vi "FuncVI_Sub - XYGraph - Master.vi"() -> ()   [LabVIEW 2021]
doc: "::: CalcExpress Toolkit :::\nCopyright (c) 2000-2026 Konstantin Shifershteyn. All rights reserved."
panel:
  in  "data":string
  in  "update":bool
  out "graph":T1(graph)
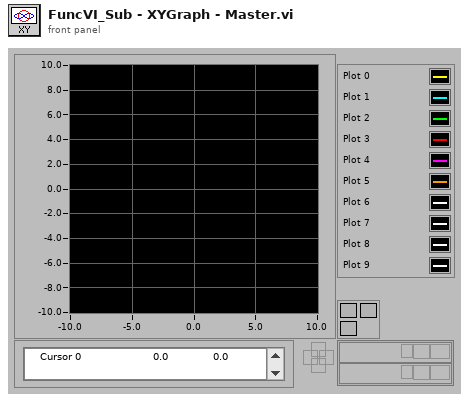
[diagram p1: front panel]
types:
  T1 = cluster{"Sine Wave":dbl[], "Sine Wave copy":dbl[]}[]
  T2 = typedef "LVRectTypeDef.ctl" = cluster{"Left":i16, "Top":i16, "Right":i16, "Bottom":i16}
  T3 = cluster{"plot":i32, "X":dbl[], "Y":dbl[], "plot name":string}
  T4 = cluster{"Sine Wave":dbl[], "Sine Wave copy":dbl[]}
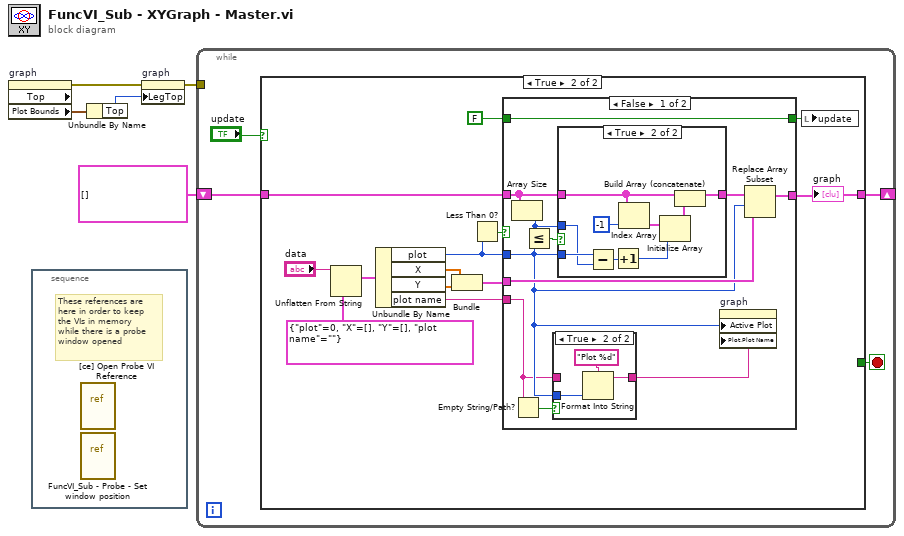
[diagram p0: block diagram]
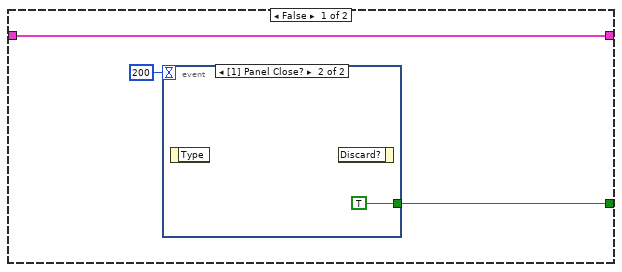
[diagram p2: hidden frame]
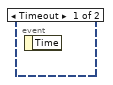
[diagram p3: hidden frame]
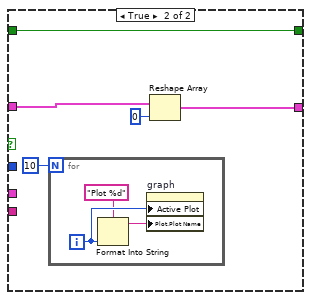
[diagram p6: hidden frame]
diagram:
  n1 = property on="graph" class="XYGraph (strict)" props=["Top", "Plot Bounds"]() -> (error out=w4:errorcluster, "Plot Bounds"=w3:T2)  [unwired: 2 in, 2 out]
  n2 = stacked-sequence {
    frame #0 {
      # "These references are\nhere in order to keep\nthe VIs in memory\nwhile there is a probe\nwindow opened"
      n3 = vi-ref "[ce] Open Probe VI Reference.vi"() -> ()  [unwired: 1 out]
      n4 = vi-ref "FuncVI_Sub - Probe - Set window position.vi"() -> ()  [unwired: 1 out]
    }
  }
  n5 = Unbundle By Name(w3) -> ("Top"=w1:i16)
  n6 = property on="graph" class="XYGraph (strict)"(error in=w4, "LegTop"=w1) -> (error out=w2:errorcluster)  [unwired: 1 in, 1 out]
  n7 = while {
    shift-right: [w7] -> _
    shift-left: T1 [] -> [w8]
    tunnel: w2 -> [_]
    stop <- w6 stop-if-true
    n8 = case shown="True" "update" {
      tunnel: w8 -> [w12 w17]
      tunnel: [w12 w16] -> w7
      tunnel: [w10 _] -> w6
      frame False {
        n9 = event shown="[1] Panel Close?" {
          selector: _ -> [_ _]
          dyn-events: _ -> [_ _]
          timeout: 200 -> [_ _]
          tunnel: [_ TRUE] -> w10
          event Timeout {
            n10 = event-data() -> ()  [unwired: 1 in, 1 out]
          }
          event Panel Close? {
            n11 = event-data() -> ()  [unwired: 1 in, 1 out]
            n12 = event-data ("Event Filter Node")() -> ()  [unwired: 2 in, 1 out]
          }
        }
      }
      frame True {
        n13 = Unflatten From String(type=T3 {"plot"=0, "X"=[], "Y"=[], "plot name"=""}, binary string="data") -> (value=w22:T3)  [unwired: 3 in, 2 out]
        n14 = Unbundle By Name(w22) -> ("plot"=w21:i32, "X"=w18:dbl[], "Y"=w19:dbl[], "plot name"=w20:string)
        n15 = Bundle("X"=w18, "Y"=w19) -> (w25:cluster{"X":dbl[], "Y":dbl[]})  [unwired: 1 in]
        n16 = Less Than 0?(x=w21) -> (x < 0?=w26:bool)
        n17 = case shown="False" w26 {
          tunnel: w21 -> [w31 _]
          tunnel: w17 -> [w36 w52]
          tunnel: [w33 w56] -> w16
          tunnel: w25 -> [w32 _]
          tunnel: w20 -> [w28 _]
          tunnel: [w27 w53] -> w15
          tunnel: FALSE ("update") -> [w27 w53]
          frame False {
            n18 = Array Size(array=w36) -> (size(s)=w35:i32)
            n19 = Empty String/Path?(string/path=w28) -> (empty?=w29:bool)
            n20 = Less Or Equal?(x=w35, y=w31) -> (x <= y?=w37:bool)
            n21 = case shown="True" w29 {
              tunnel: w31 -> [_ w40]
              tunnel: [w38 w39] -> w30
              tunnel: w28 -> [w38 _]
              frame False {
              }
              frame True {
                n22 = Format Into String(format string="Plot %d", w40) -> (resulting string=w39:string)  [unwired: 2 in, 1 out]
              }
            }
            n23 = case shown="True" w37 {
              tunnel: w36 -> [w42 w45]
              tunnel: w31 -> [_ w51]
              tunnel: [w42 w46] -> w34
              tunnel: w35 -> [_ w50]
              frame False {
              }
              frame True {
                n24 = Subtract(x=w51, y=w50) -> (x-y=w49:i32)
                n25 = Increment(x=w49) -> (x+1=w48:i32)
                n26 = Index Array(array=w45, index=-1) -> (element=w44:T4)
                n27 = Initialize Array(w44, w48) -> (w47:T1)
                n28 = Build Array (concatenate)(w45, w47) -> (w46:T1)
              }
            }
            n29 = property on="graph" class="XYGraph (strict)"("Active Plot"=w31, "Plot.Plot Name"=w30) -> ()  [unwired: 2 in, 2 out]
            n30 = Replace Array Subset(array=w34, new element=w32, index=w31) -> (w33:T1)
          }
          frame True {
            n31 = for {
              N: 10 -> [_]
              i -> [w58]
              n32 = Format Into String(format string="Plot %d", w58) -> (resulting string=w59:string)  [unwired: 2 in, 1 out]
              n33 = property on="graph" class="XYGraph (strict)"("Active Plot"=w58, "Plot.Plot Name"=w59) -> ()  [unwired: 2 in, 2 out]
            }
            n34 = Reshape Array(w52, 0) -> (w56:T1)
          }
        }
        "graph" <- w16
        n35 = local write "update"(w15) -> ()
      }
    }
  }
